vi "labels.set.vi"(8 "error in":errorcluster, 10 "Labels":string[](array[string]), 11 "asset in":refnum<class "asset.lvclass">) -> (0 "error out":errorcluster, 3 "asset out":refnum<class "asset.lvclass">)   [LabVIEW 2020, in "asset.lvclass"]
uses:
  asset.lvclass
  asset.lvclass/asset.ctl
  Nominal Client/Nominal Client.lvclass
  <vilib>/JDP Science/JSONtext/JSONtext.lvlib
  nominal types/labels/labels.lvclass
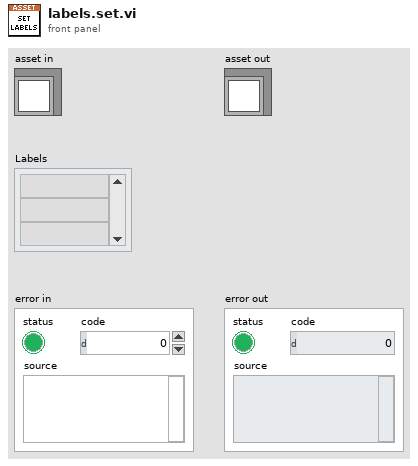
[diagram p1: front panel]
types:
  T1 = typedef "dataScopes.lvlib/links.ctl" = cluster{"URL":string, "Title":string}[]
  T2 = typedef "dataScopes.lvlib/data_scopes.ctl" = T3[]
  T3 = typedef "dataScopes.lvlib/data_scope.ctl" = cluster{"dataScopeName":string, "dataSource":T4, "seriesTags":refnum<class "properties.lvclass">, "offset":T6}
  T4 = typedef "dataScopes.lvlib/data_source.ctl" = cluster{"type":T5, "rid":string}
  T5 = typedef "dataScopes.lvlib/type.ctl" = enum16{"dataset", "connection", "logSet", "video"}
  T6 = typedef "dataScopes.lvlib/offset.ctl" = cluster{"seconds":i32, "nanos":i32, "picos":i32}
  T7 = cluster{"rid":string, "title":string, "properties":refnum<class "properties.lvclass">, "labels":refnum<class "labels.lvclass">, "Links":T1, "datascopes":T2, "createdAt":timestamp, "updatedAt":timestamp, "attachments":refnum<class "labels.lvclass">, "isStaged":bool, "isArchived":bool, "description":string, "createdBy":string, "type":string}
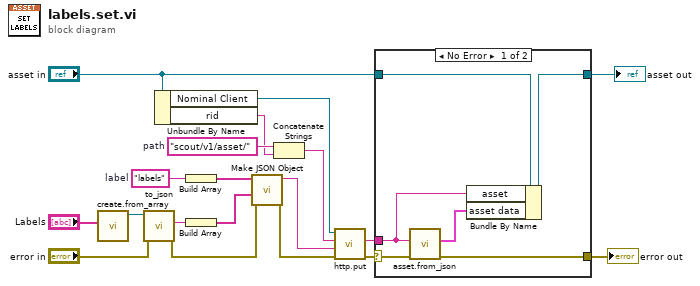
[diagram p0: block diagram]
diagram:
  w8 = "labels"  # label
  w18 = "scout/v1/asset/"  # path
  n1 = call "create.from_array.vi"("labels"="Labels") -> ("labels out"=w2:refnum<class "labels.lvclass">)  [unwired: 10 in]
  n2 = call-dynamic "to_json.vi"("error in"="error in", "labels in"=w2) -> ("error out"=w3:errorcluster, "json"=w5:string)  [unwired: 6 in, 2 out]
  n3 = Unbundle By Name("asset in") -> ("Nominal Client"=w19:refnum<class "Nominal Client.lvclass">, "rid"=w16:string)
  n4 = Build Array(w8) -> (w9:string[])
  n5 = Build Array(w5) -> (w10:string[])
  n6 = call <vilib>:"Make JSON Object.vi"("error in (no error)"=w3, "JSON Items"=w10, "Item Names"=w9) -> ("error out"=w6:errorcluster, "<JSON>"=w7:string)  [unwired: 7 in]
  n7 = Concatenate Strings(w18, w16) -> (w17:string)
  n8 = call "http.put.vi"("error in"=w6, "Body"=w7, "Path"=w17, "Nominal Client in"=w19) -> ("error out"=w15:errorcluster, "Response"=w12:string)  [unwired: 4 in, 2 out]
  n9 = case shown="No Error" w15 {
    selector: w15 -> [w25 w27]
    tunnel: [w24 w27] -> w14
    tunnel: "asset in" -> [w23 w26]
    tunnel: w12 -> [w21 _]
    tunnel: [w20 w26] -> w11
    frame No Error {
      n10 = call "asset.from_json.vi"("error in"=w25, "asset"=w21) -> ("error out"=w24:errorcluster, "Asset Data"=w22:T7)  [unwired: 8 in]
      n11 = Bundle By Name(cluster=w23, "asset"=w21, "asset data"=w22) -> (w20:refnum<class "asset.lvclass">)
    }
    frame Error {
    }
  }
  "asset out" <- w11
  "error out" <- w14
